vi "libssh2_knownhost_init.vi"(8 "error in (no error)":errorcluster, 11 "session":T1) -> (0 "error out":errorcluster, 3 "host key database":T2)   [LabVIEW 2017, in "libssh2.lvlib"]
doc: "Initialize a host key database."
uses:
  libssh2.lvlib
  Host Key Database Refnum.ctl
  Session Refnum.ctl
  Not A Session.vi
  <vilib>/Utility/error.llb/Error Cluster From Error Code.vi
  Global Settings.vi
  Read Session Refnum.vi
  <vilib>/Utility/semaphor.llb/Acquire Semaphore.vi
  <vilib>/Utility/semaphor.llb/Release Semaphore.vi
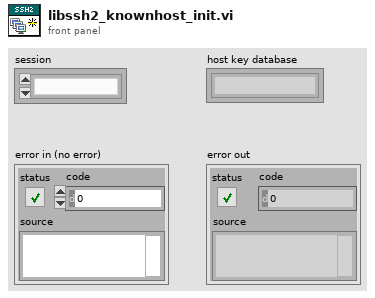
[diagram p1: front panel]
types:
  T1 = typedef "libssh2.lvlib/Session Refnum.ctl" = refnum<k1>
  T2 = typedef "libssh2.lvlib/Host Key Database Refnum.ctl" = refnum<k1>
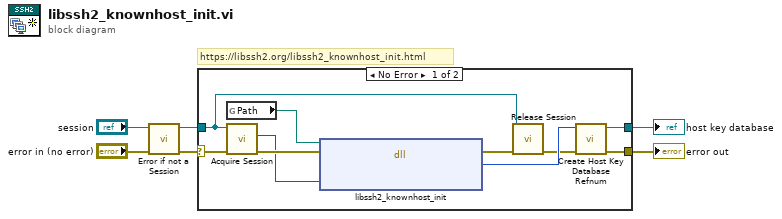
[diagram p0: block diagram]
diagram:
  # "https://libssh2.org/libssh2_knownhost_init.html"
  n1 = call "Error if not a Session.vi"("error in (no error)"="error in (no error)", "session"="session") -> ("error out"=w3:errorcluster, "session out"=w1:T1)  [unwired: 8 in]
  n2 = case shown="No Error" w3 {
    selector: w3 -> [w14 w17]
    tunnel: w1 -> [w7 _]
    tunnel: [w16 w17] -> w6
    tunnel: [w15 _] -> w5
    frame No Error {
      n3 = global read "Global Settings.vi" "Path"() -> (w9:path)
      n4 = call "Acquire Session.vi"("error in (no error)"=w14, "session"=w7) -> ("error out"=w12:errorcluster, "LIBSSH2_SESSION*"=w11:u64)  [unwired: 7 in, 1 out]
      n5 = dll-call lib="?" fn="libssh2_knownhost_init"(path in=w9, error in=w12, "session"=w11) -> (error out=w13:errorcluster, "return value"=w10:u64)  [unwired: 2 in, 1 out]
      n6 = call "Release Session.vi"("error in (no error)"=w13, "session"=w7) -> ("error out"=w8:errorcluster)  [unwired: 9 in]
      n7 = call "Create Host Key Database Refnum.vi"("error in (no error)"=w8, "LIBSSH2_KNOWNHOSTS*"=w10) -> ("error out"=w16:errorcluster, "host key database"=w15:T2)  [unwired: 8 in]
    }
    frame Error {
    }
  }
  "host key database" <- w5
  "error out" <- w6
